vi "RemoteVI Open URL.vi"(0 "URL":string) -> (15 "error out":errorcluster)   [LabVIEW 2020, in "RemoteVI.lvlib"]
doc: "Opens URL in the default web browser (rundll32 url.dll,FileProtocolHandler, through System Exec.vi, without waiting). RemoteVI Server's Open in browser."
uses:
  RemoteVI.lvlib
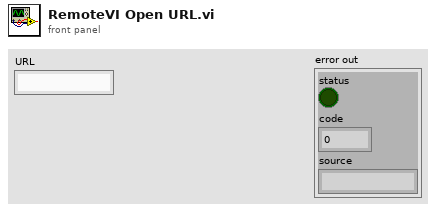
[diagram p1: front panel]
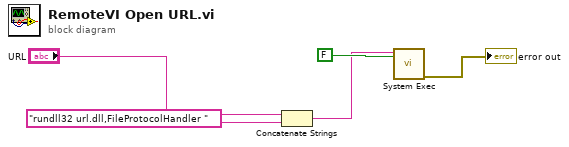
[diagram p0: block diagram]
diagram:
  n1 = Concatenate Strings("rundll32 url.dll,FileProtocolHandler ", "URL") -> (w3:string)
  n2 = call <vilib>:"System Exec.vi"("wait until completion? (T)"=FALSE, "command line"=w3) -> ("error out"=→"error out":errorcluster)  [unwired: 6 in, 3 out]
